vi "Are All Indexes In Range (1D Array).vi"(1 "Array of Indexes":i32[](array[numeric]), 2 "Array Number of Elements (Array Size)":i32) -> (0 "Are All Indexes In Range?":bool)   [LabVIEW 2026, in "RSysUtils Array.lvlib"]
doc: "This VI checks whether all indexes in an array are inside the range of an Array (whether they are valid indexes to index out of an array).\nThis VI outputs True if and only if all indexes have a value between 0 and \"Array Number of Elements - 1\".\nSpecial cases:\n - Outputs True if the \"Array of Indexes\" is empty, regardless of the \"Array Number of Elements\""
uses:
  RSysUtils Array.lvlib
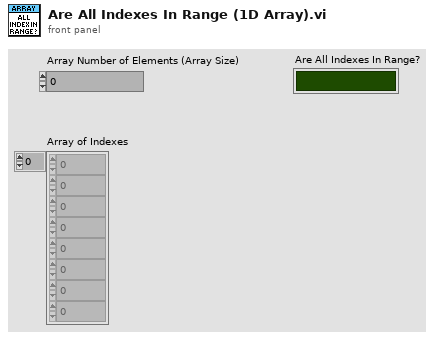
[diagram p1: front panel]
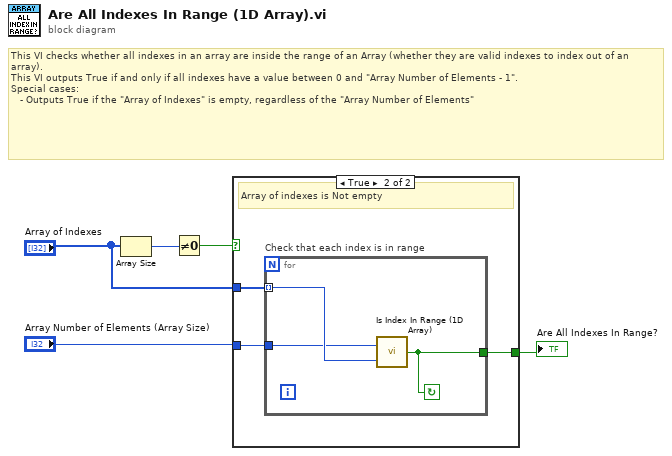
[diagram p0: block diagram]
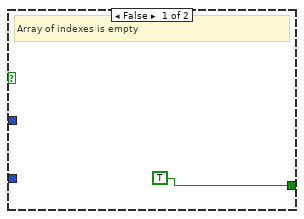
[diagram p2: hidden frame]
diagram:
  # "This VI checks whether all indexes in an array are inside the range of an Array (whether they are valid indexes to index out of an array).\nThis VI outputs True if and only if all indexes have a value between 0 and \"Array Number of Elements - 1\".\nSpecial cases:\n   - Outputs True if the \"Array of Indexes\" is empty, regardless of the \"Array Number of Elements\""
  n1 = Array Size(array="Array of Indexes") -> (size(s)=w5:i32)
  n2 = Not Equal To 0?(x=w5) -> (x != 0?=w4:bool)
  n3 = case shown="True" w4 {
    tunnel: [TRUE w8] -> w3
    tunnel: "Array of Indexes" -> [_ w9]
    tunnel: "Array Number of Elements (Array Size)" -> [_ w7]
    frame False {
      # "Array of indexes is empty"
    }
    frame True {
      # "Array of indexes is Not empty"
      n4 = for "Check that each index is in range" {
        tunnel: w9 -> [w12] mode=indexing
        tunnel: [w10] -> w8
        tunnel: w7 -> [w11]
        stop <- w10 continue-if-true
        n5 = call "Is Index In Range (1D Array).vi"("Index"=w12, "Array Number of Elements (Array Size)"=w11) -> ("Is Index In Range?"=w10:bool)
      }
    }
  }
  "Are All Indexes In Range?" <- w3
